vi "sema.vi"() -> ()   [LabVIEW 2013]
panel:
  out "Trajanje":dbl
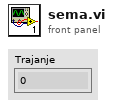
[diagram p1: front panel]
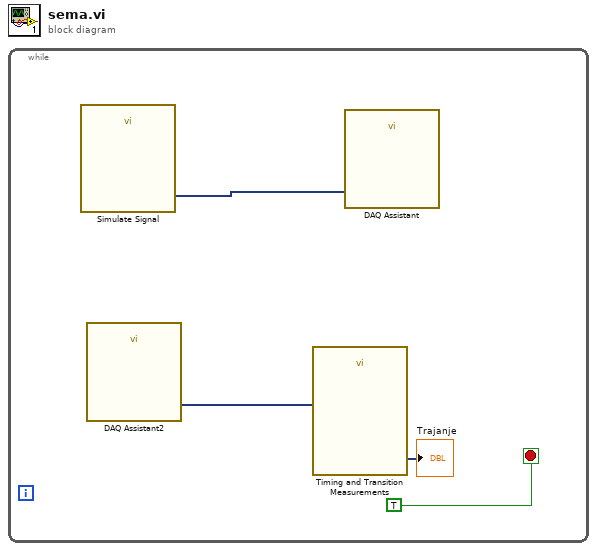
[diagram p0: block diagram]
diagram:
  n1 = while {
    stop <- TRUE stop-if-true
    n2 = call "Simulate Signal"() -> ("Square"=w3:dynamicdata)  [unwired: 14 in, 1 out]
    n3 = call "DAQ Assistant2"() -> ("data"=w2:dynamicdata)  [unwired: 16 in, 3 out]
    n4 = call "Timing and Transition Measurements"("Signals"=w2) -> ("Duration"=→"Trajanje":dynamicdata)  [unwired: 9 in, 1 out]
    n5 = call "DAQ Assistant"("data"=w3) -> ()  [unwired: 16 in, 3 out]
  }
